vi "AutoMapVIs.vi"(5 "Ignore if Not Found?":bool, 6 "Payload":string, 7 "SubPanel in":refnum<vi>, 8 "error in (no error)":errorcluster, 9 "Command":string, 10 "VI Paths":path[](array[path]), 11 "Fully Qualified VI Names":string[](array[string])) -> (0 "error out":errorcluster, 2 "Response":string, 3 "Match Present?":bool)   [LabVIEW 2019, in "MicronServer.lvlib" / "Mapper.lvclass"]
uses:
  Mapper.lvclass
  <vilib>/LabJSON/Typedefs/Settings.ctl
  841f89ec-ee0f-447c-a6b4-e789bd2a3d19.vi
  3509af77-3f70-4233-9ace-5198743abfec.vi
  b42673da-ce77-4f84-840a-27f1bd3cdd3a.vi
  <vilib>/LabJSON/APIs/RunVIRefnum.vi
  <vilib>/JDP Science/JSONtext/Variant to JSON Text.vi
  <vilib>/JDP Science/JSONtext/support/Format JSON Object.vi
  <vilib>/JDP Science/JSONtext/LVClass Serializer/JSONtext LVClass Serializer.lvclass
  <vilib>/LabJSON/LabJSON.lvlib
  <vilib>/JDP Science/JSONtext/JSONtext.lvlib
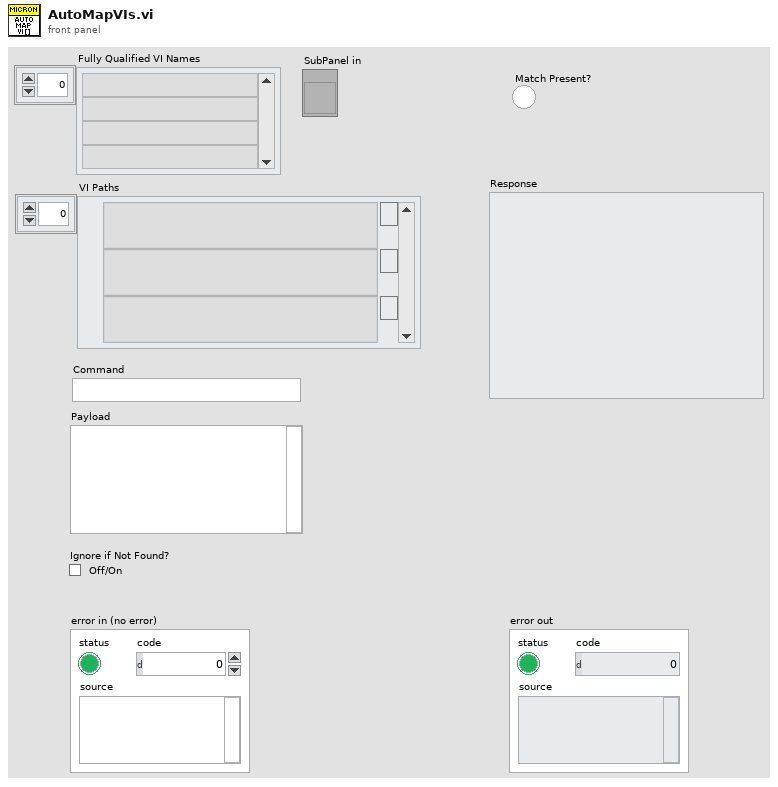
[diagram p1: front panel]
types:
  T1 = typedef "LabJSON.lvlib/Settings.ctl" = cluster{"Reinitialize to Default?":bool, "Show Front Panel?":bool, "Close Front Panel?":bool, "Ignore if Not Found?":bool}
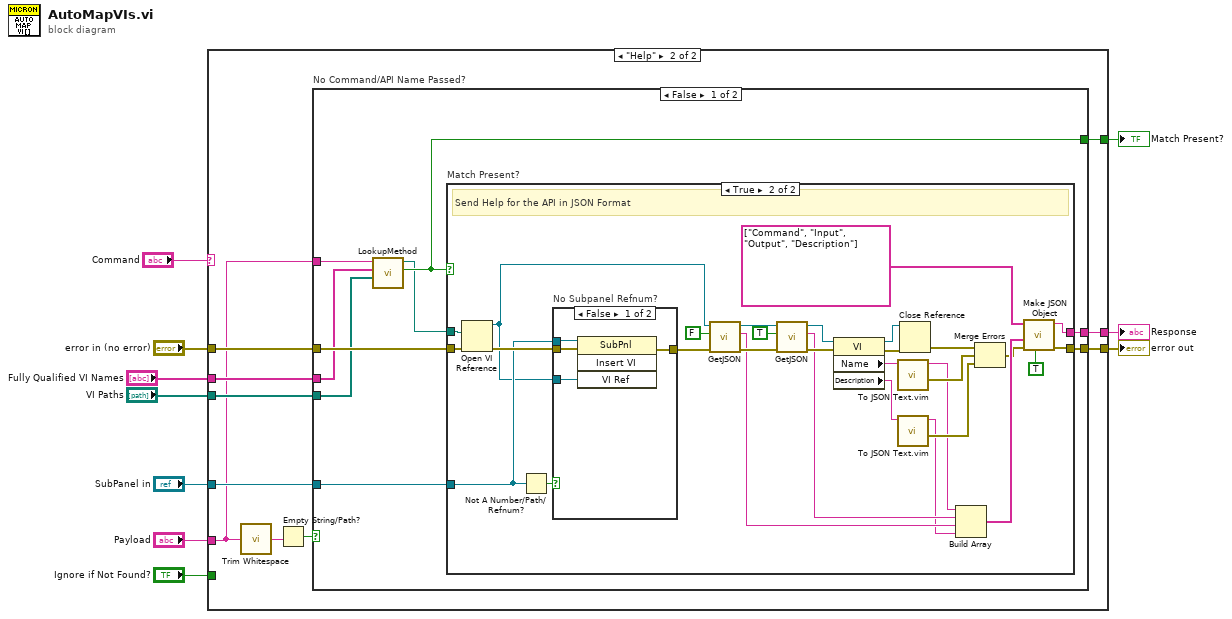
[diagram p0: block diagram]
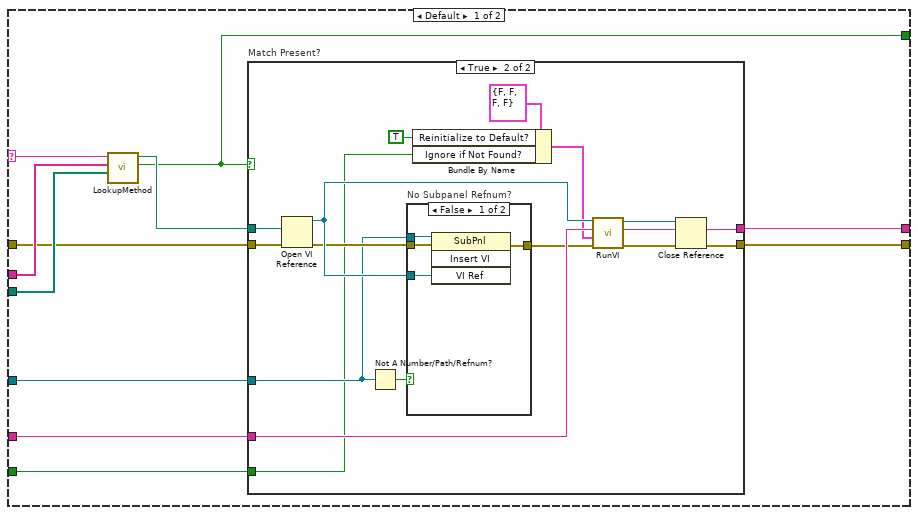
[diagram p2: hidden frame]
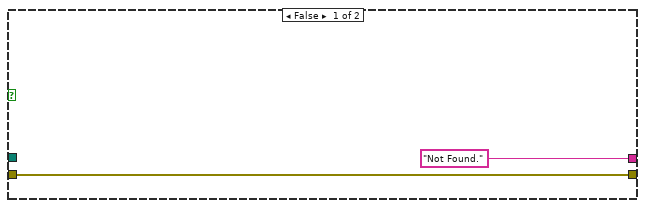
[diagram p5: hidden frame]
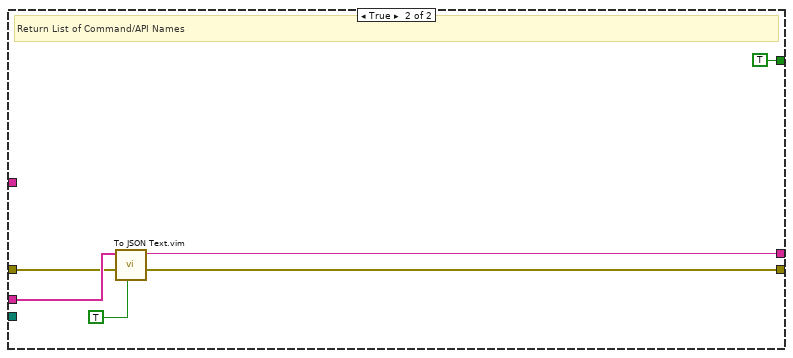
[diagram p7: hidden frame]
diagram:
  n1 = case shown="\"Help\"" "Command" {
    selector: "Command" -> [w19 _]
    tunnel: "Fully Qualified VI Names" -> [w21 w53]
    tunnel: "VI Paths" -> [w20 w52]
    tunnel: "Payload" -> [w18 w46]
    tunnel: [w17 w51] -> w5
    tunnel: "SubPanel in" -> [w15 w50]
    tunnel: "error in (no error)" -> [w14 w49]
    tunnel: [w13 w48] -> w8
    tunnel: [w12 w47] -> w9
    tunnel: "Ignore if Not Found?" -> [w11 _]
    frame Default {
      n2 = call "LookupMethod.vi"("Method Paths"=w20, "Fully Qualified Method Names"=w21, "Command"=w19) -> ("Found?"=w12:bool, "Method Path"=w16:path)  [unwired: 7 in]
      n3 = case "Match Present?" shown="True" w12 {
        tunnel: w18 -> [_ w38]
        tunnel: [_ w37] -> w17
        tunnel: w16 -> [_ w36]
        tunnel: w15 -> [_ w27]
        tunnel: w14 -> [w22 w31]
        tunnel: [w22 w25] -> w13
        tunnel: w11 -> [_ w23]
        frame False {
        }
        frame True {
          n4 = Open VI Reference(vi path=w36, error in (no error)=w31) -> (vi reference=w35:refnum<vi>, error out=w30:errorcluster)  [unwired: 4 in]
          n5 = Not A Number/Path/Refnum?(number/path/refnum=w27) -> (NaN/Path/Refnum?=w26:bool)
          n6 = case "No Subpanel Refnum?" shown="False" w26 {
            tunnel: w35 -> [w42 _]
            tunnel: w30 -> [w41 w43]
            tunnel: [w40 w43] -> w29
            tunnel: w27 -> [w39 _]
            frame False {
              n7 = invoke class="SubPnl" method="Insert VI"(reference=w39, error in=w41, "VI Ref"=w42) -> (error out=w40:errorcluster)  [unwired: 1 in, 3 out]
            }
            frame True {
            }
          }
          n8 = Bundle By Name(cluster=T1 {"Reinitialize to Default?"=FALSE, "Show Front Panel?"=FALSE, "Close Front Panel?"=FALSE, "Ignore if Not Found?"=FALSE} ("Settings"), "Reinitialize to Default?"=TRUE, "Ignore if Not Found?"=w23) -> (w33:T1)
          n9 = call-poly <vilib>:"RunVI.vi"("Error In"=w29, "Settings"=w33, "JSON Input"=w38, "VI Refnum In"=w35) -> ("Error Out"=w28:errorcluster, "JSON Output"=w37:string, "VI Refnum Out"=w24:refnum<vi>)  [unwired: 5 in]
          n10 = Close Reference(reference=w24, error in (no error)=w28) -> (error out=w25:errorcluster)
        }
      }
    }
    frame "Help" {
      n11 = call <vilib>:"Trim Whitespace.vi"("string"=w46) -> ("trimmed string"=w45:string)  [unwired: 1 in]
      n12 = Empty String/Path?(string/path=w45) -> (empty?=w44:bool)
      n13 = case "No Command/API Name Passed?" shown="False" w44 {
        tunnel: w53 -> [w57 w105]
        tunnel: w52 -> [w56 _]
        tunnel: [w62 w101] -> w51
        tunnel: w50 -> [w61 _]
        tunnel: w49 -> [w60 w104]
        tunnel: [w59 w103] -> w48
        tunnel: [w55 TRUE] -> w47
        tunnel: w46 -> [w58 _]
        frame False {
          n14 = call "LookupMethod.vi"("Method Paths"=w56, "Fully Qualified Method Names"=w57, "Command"=w58) -> ("Found?"=w55:bool, "Method Path"=w54:path)  [unwired: 7 in]
          n15 = case "Match Present?" shown="True" w55 {
            tunnel: ["Not Found." ("JSON Output") w82] -> w62
            tunnel: w54 -> [_ w94]
            tunnel: w61 -> [_ w91]
            tunnel: w60 -> [w64 w93]
            tunnel: [w64 w84] -> w59
            frame False {
            }
            frame True {
              # "Send Help for the API in JSON Format"
              n16 = Open VI Reference(vi path=w94, error in (no error)=w93) -> (vi reference=w88:refnum<vi>, error out=w92:errorcluster)  [unwired: 4 in]
              n17 = Not A Number/Path/Refnum?(number/path/refnum=w91) -> (NaN/Path/Refnum?=w90:bool)
              n18 = case "No Subpanel Refnum?" shown="False" w90 {
                tunnel: w88 -> [w98 _]
                tunnel: w92 -> [w97 w99]
                tunnel: [w96 w99] -> w89
                tunnel: w91 -> [w95 _]
                frame False {
                  n19 = invoke class="SubPnl" method="Insert VI"(reference=w95, error in=w97, "VI Ref"=w98) -> (error out=w96:errorcluster)  [unwired: 1 in, 3 out]
                }
                frame True {
                }
              }
              n20 = call <vilib>:"GetJSON.vi"("Error In"=w89, "Controls?"=FALSE, "VI Refnum In"=w88) -> ("Error Out"=w78:errorcluster, "JSON Out"=w72:string, "VI Refnum Out"=w76:refnum<vi>)  [unwired: 6 in]
              n21 = call <vilib>:"GetJSON.vi"("Error In"=w78, "Controls?"=TRUE, "VI Refnum In"=w76) -> ("Error Out"=w77:errorcluster, "JSON Out"=w73:string, "VI Refnum Out"=w74:refnum<vi>)  [unwired: 6 in]
              n22 = property class="VI"(reference=w74, error in=w77) -> (reference out=w85:refnum<vi>, error out=w86:errorcluster, "Name"=w71:string, "Description"=w70:string)
              n23 = call "To JSON Text.vim"("Anything"=w71) -> ("error out"=w68:errorcluster, "<JSON>"=w66:string)  [unwired: 9 in]
              n24 = call "To JSON Text.vim"("Anything"=w70) -> ("error out"=w67:errorcluster, "<JSON>"=w65:string)  [unwired: 9 in]
              n25 = Close Reference(reference=w85, error in (no error)=w86) -> (error out=w81:errorcluster)
              n26 = Build Array(w66, w73, w72, w65) -> (w80:string[])
              n27 = Merge Errors(w81, w68, w67) -> (w69:errorcluster)
              n28 = call <vilib>:"Make JSON Object.vi"("Pretty Print?"=TRUE, "error in (no error)"=w69, "JSON Items"=w80, "Item Names"=string[] ["Command", "Input", "Output", "Description"]) -> ("error out"=w84:errorcluster, "<JSON>"=w82:string)  [unwired: 6 in]
            }
          }
        }
        frame True {
          # "Return List of Command/API Names"
          n29 = call "To JSON Text.vim"("Pretty Print?"=TRUE, "error in (no error)"=w104, "Anything"=w105) -> ("error out"=w103:errorcluster, "<JSON>"=w101:string)  [unwired: 7 in]
        }
      }
    }
  }
  "Match Present?" <- w9
  "error out" <- w8
  "Response" <- w5
